vi "Write Index.vi"(8 "error in (no error)":errorcluster, 10 "index":i32, 11 "NT Enum in":refnum<class "NT Enum.lvclass">) -> (0 "error out":errorcluster, 3 "NT Enum out":refnum<class "NT Enum.lvclass">)   [LabVIEW 2020, in "PV Access.lvlib" / "PV Data.lvlib" / "NT Enum.lvclass"]
uses:
  NT Enum.lvclass
  NT Enum.lvclass/NT Enum.ctl
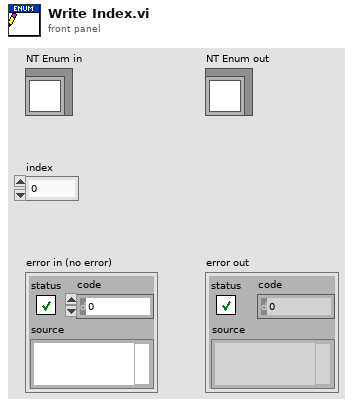
[diagram p1: front panel]
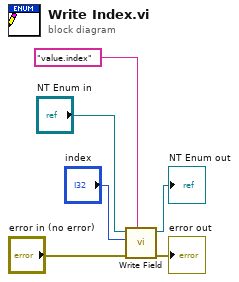
[diagram p0: block diagram]
diagram:
  n1 = call-dynamic "Write Field.vi"("field"="value.index", "error in (no error)"="error in (no error)", "value"="index", "Base Interface in"="NT Enum in") -> ("error out"=→"error out":errorcluster, "Base Interface out"=→"NT Enum out":refnum<class "NT Enum.lvclass">)  [unwired: 6 in]
